vi "Send Stream Event.vi"(8 "error in":errorcluster, 9 "send?":bool, 10 "event":string, 11 "events":refnum<queue>) -> (0 "error out":errorcluster, 3 "client gone?":bool)   [LabVIEW 2020, in "MCP Server.lvlib"]
doc: "When send? is TRUE, puts one Server-Sent Event on the events queue of the streamed tools/call and waits up to 1 s for the stream to take it (Wait For Stream Drain.vi). client gone? is TRUE when it was not taken: the client has closed the stream, which is how a client cancels over HTTP. Used by Report Progress.vi (progress notifications) and Cancel Requested.vi (keep-alive probes).\n\nWhen send? is FALSE nothing is sent and client gone? is FALSE. Runs regardless of error in, which is passed through unchanged; queue errors count as not taken and are not passed on."
uses:
  MCP Server.lvlib
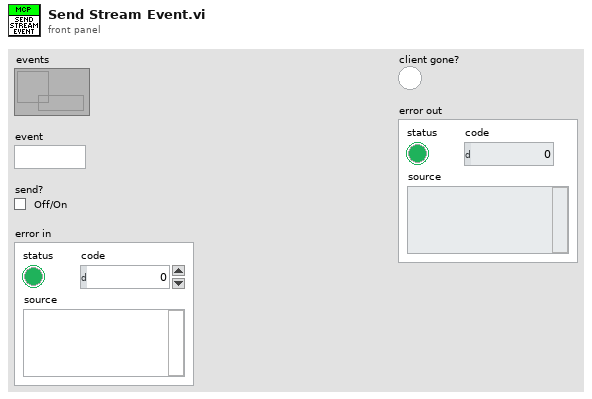
[diagram p1: front panel]
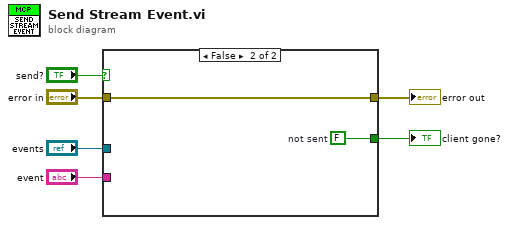
[diagram p0: block diagram]
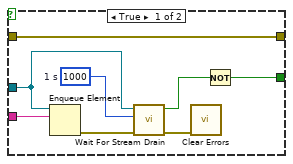
[diagram p2: hidden frame]
diagram:
  n1 = case shown="False" "send?" {
    tunnel: "events" -> [w13 _]
    tunnel: "event" -> [w14 _]
    tunnel: "error in" -> [w7 w15]
    tunnel: [w8 w16] -> w2
    tunnel: [w7 w15] -> w1
    frame True {
      w12 = 1000  # 1 s
      n2 = Enqueue Element(queue=w13, element=w14) -> (error out=w11:errorcluster)  [unwired: 2 in, 2 out]
      n3 = call "Wait For Stream Drain.vi"("error in"=w11, "timeout ms"=w12, "events"=w13) -> ("error out"=w10:errorcluster, "drained?"=w9:bool)  [unwired: 7 in]
      n4 = call <vilib>:"Clear Errors.vi"("error in (no error)"=w10) -> ()  [unwired: 5 in, 2 out]
      n5 = Not(x=w9) -> (.not. x?=w8:bool)
    }
    frame False {
      w16 = FALSE  # not sent
    }
  }
  "client gone?" <- w2
  "error out" <- w1
